vi "PicoScope5000aOpen.vi"(0 "error in (no error)":errorcluster, 1 "Serial Number":string, 2 "Mode":u16(ring) items=["Dialog On Error", "no dialog - CloseUnit and Stop", "no dialog - Continue", "no dialog - Stop"], 5 "Use Serial Number":bool, 9 "Resolution":u32(ring) items=["8-bit", "12-bit", "14-bit", "15-bit (max. 2 ch.)", "16-bit (max. 1 ch.)"], 11 "USB Powered control":bool=TRUE, 15 "USB 3.0 device on non-USB 3.0 Port control":bool=TRUE) -> (3 "USB 3.0 device on non-USB 3.0 Port":bool=TRUE, 4 "error out":errorcluster, 6 "handle":i16, 10 "USB Powered":bool=TRUE, 12 "Device Info":T1, 14 "Max ADC value":i16)   [LabVIEW 2010]
doc: "This VI opens a PicoScope ps5000a API device and returns a handle to the device."
uses:
  ps5000a.dll
panel:
  out "count":i16
  out "serialLth":i16
  out "Pico 5000a Units":string
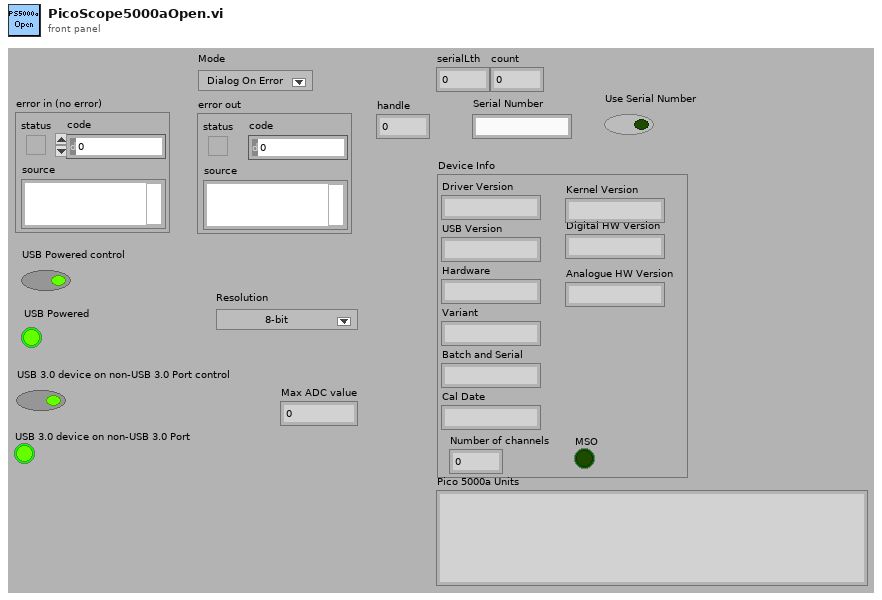
[diagram p1: front panel]
types:
  T1 = cluster{"Driver Version":string, "USB Version":string, "Hardware":string, "Variant":string, "Batch and Serial":string, "Cal Date":string, "Kernel Version":string, "Digital HW Version":string, "Analogue HW Version":string, "MSO":bool, "Number of channels":i16}
  T2 = cluster{"status":bool, "code":u32, "source":string}
  T3 = cluster{"Driver Version":string, "USB Version":string, "Hardware":string, "Variant":string, "Batch and Serial":string, "Cal Date":string, "Kernel Version":string, "Digital HW Version":string, "Analogue HW Version":string, "Firmware 1":string, "Firmware 2":string}
  T4 = cluster{"Driver Version":string, "USB Version":string, "Hardware":string, "Variant":string, "Batch and Serial":string, "Cal Date":string, "Kernel Version":string, "Digital HW Version":string, "Analogue HW Version":string, bool, i16}
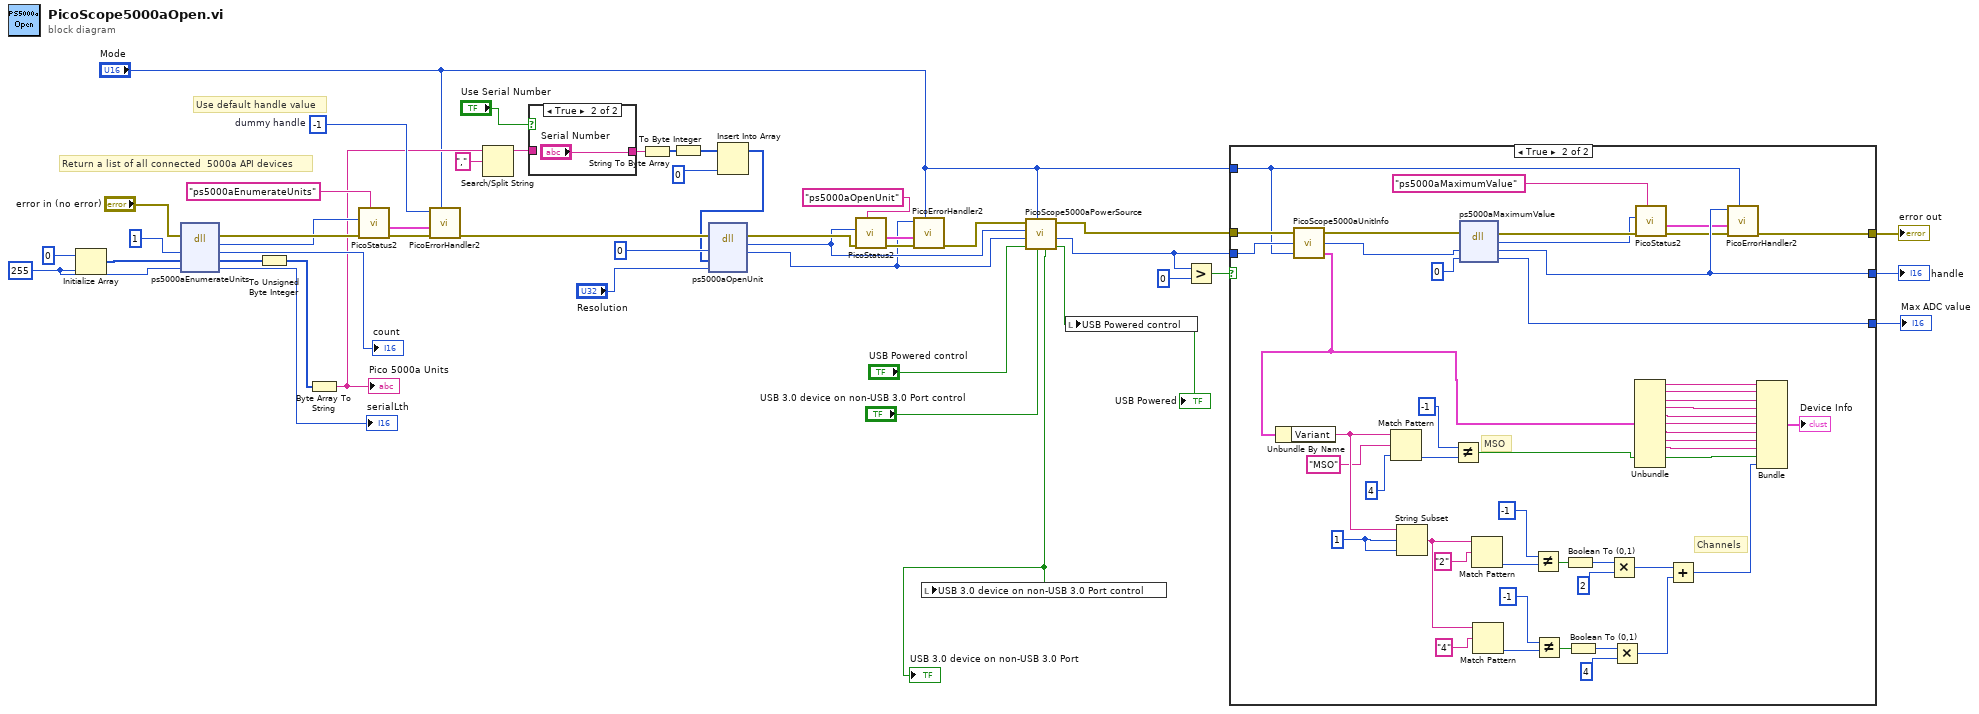
[diagram p0: block diagram]
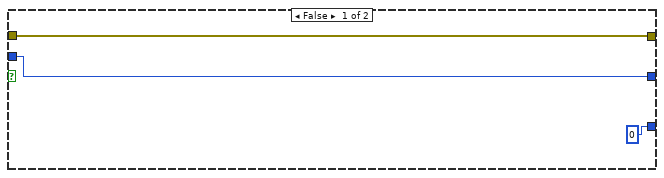
[diagram p3: hidden frame]
diagram:
  w26 = i16 -1  # dummy handle
  w29 = i16 255 ("dimension size")
  # "Use default handle value"
  # "Return a list of all connected  5000a API devices"
  n1 = Initialize Array(i8 0 ("U8"), w29) -> (w31:i8[])
  n2 = dll-call lib="ps5000a.dll" fn="ps5000aEnumerateUnits"(error in="error in (no error)", "count"=i16 1, "serials"=w31, "serialLth"=w29) -> (error out=w23:errorcluster, "PICO_STATUS"=w21:u32, "count"=→"count":i16, "serials"=w27:i8[], "serialLth"=→"serialLth":i16)  [unwired: 2 in, 1 out]
  n3 = To Unsigned Byte Integer(number=w27) -> (unsigned 8bit integer=w28:u8[])
  n4 = Byte Array To String(unsigned byte array=w28) -> (string=w15:string)
  "Pico 5000a Units" <- w15
  n5 = call "PicoStatus2.vi"("PICO source"="ps5000aEnumerateUnits" ("source"), "Error in"=w23, "PICO STATUS"=w21) -> ("error out"=w25:errorcluster, "PICO_STATUS out"=w24:T2)  [unwired: 5 in]
  n6 = call "PicoErrorHandler2.vi"("Mode"="Mode", "error in (no error)"=w25, "PICO_STATUS in"=w24, "handle In"=w26) -> ("error out"=w35:errorcluster)  [unwired: 7 in]
  n7 = Search/Split String(string=w15, search string/char (-)=",") -> (substring before match=w13:string)  [unwired: 1 in, 2 out]
  n8 = case shown="True" "Use Serial Number" {
    tunnel: w13 -> [w47 _]
    tunnel: [w47 "Serial Number"] -> w9
    frame False {
    }
    frame True {
    }
  }
  n9 = String To Byte Array(string=w9) -> (unsigned byte array=w11:u8[])
  n10 = To Byte Integer(number=w11) -> (8bit integer=w12:i8[])
  n11 = Insert Into Array(array=w12, new element=i8 0 ("new element/subarray")) -> (w8:i8[])  [unwired: 1 in]
  n12 = dll-call lib="ps5000a.dll" fn="ps5000aOpenUnit" ("ps3000.dll:_ps3000_open_unit@0")(error in=w35, "handle"=i16 0, "serial"=w8, "resolution"="Resolution") -> (error out=w18:errorcluster, "PICO_STATUS"=w3:u32, "handle"=w2:i16)  [unwired: 4 in, 1 out]
  n13 = call "PicoStatus2.vi"("PICO source"="ps5000aOpenUnit" ("source"), "Error in"=w18, "PICO STATUS"=w3) -> ("error out"=w17:errorcluster, "PICO_STATUS out"=w20:T2)  [unwired: 5 in]
  n14 = call "PicoErrorHandler2.vi"("Mode"="Mode", "error in (no error)"=w17, "PICO_STATUS in"=w20, "handle In"=w2) -> ("error out"=w4:errorcluster)  [unwired: 7 in]
  n15 = call "PicoScope5000aPowerSource.vi"("USB 3.0 on non-USB 3.0 port control"="USB 3.0 device on non-USB 3.0 Port control", "Mode"="Mode", "USB Powered control"="USB Powered control", "handle in"=w2, "PICO STATUS IN"=w3, "error in (no error)"=w4) -> ("USB Powered"=w45:bool, "handle out"=w43:i16, "error out"=w38:errorcluster, "USB 3.0 on non-USB 3.0 Port"=w39:bool)  [unwired: 1 in, 1 out]
  "USB Powered" <- w45
  "USB 3.0 device on non-USB 3.0 Port" <- w39
  n16 = local write "USB 3.0 device on non-USB 3.0 Port control"(w39) -> ()
  n17 = local write "USB Powered control"(w45) -> ()
  n18 = Greater?(x=w43, y=0) -> (0:w44:bool)
  n19 = case shown="True" w44 {
    tunnel: w43 -> [w50 w99]
    tunnel: w38 -> [w51 w98]
    tunnel: [w51 w60] -> w36
    tunnel: [w50 w59] -> w37
    tunnel: [i16 0 ("value") w61] -> w41
    tunnel: "Mode" -> [_ w52]
    frame False {
    }
    frame True {
      w88 = 1 ("offset (0)")
      # "MSO"
      # "Channels"
      n20 = call "PicoScope5000aUnitInfo.vi"("Mode"=w52, "handle in"=w99, "error in (no error)"=w98) -> ("Unit Info"=w64:T3, "handle out"=w63:i16, "error out"=w54:errorcluster)
      n21 = Unbundle By Name(w64) -> ("Variant"=w84:string)
      n22 = Match Pattern(string=w84, regular expression="MSO", offset (0)=4) -> (offset past match=w81:i32)  [unwired: 3 out]
      n23 = String Subset(string=w84, offset (0)=w88, length (rest)=w88) -> (substring=w75:string)
      n24 = Not Equal?(x=-1, y=w81) -> (x != y?=w79:bool)
      n25 = dll-call lib="ps5000a.dll" fn="ps5000aMaximumValue"(error in=w54, "handle"=w63, "value"=i16 0) -> (error out=w57:errorcluster, "PICO_STATUS"=w55:u32, "handle"=w59:i16, "value"=w61:i16)  [unwired: 2 in, 1 out]
      n26 = Match Pattern(string=w75, regular expression="2") -> (offset past match=w86:i32)  [unwired: 1 in, 3 out]
      n27 = Match Pattern(string=w75, regular expression="4") -> (offset past match=w77:i32)  [unwired: 1 in, 3 out]
      n28 = Not Equal?(x=-1, y=w86) -> (x != y?=w71:bool)
      n29 = Not Equal?(x=-1, y=w77) -> (x != y?=w67:bool)
      n30 = Boolean To (0,1)(Boolean=w71) -> (0, 1=w70:i16)
      n31 = Boolean To (0,1)(Boolean=w67) -> (0, 1=w68:i16)
      n32 = Multiply(x=w70, y=i16 2) -> (x*y=w74:i16)
      n33 = Multiply(x=w68, y=i16 4) -> (x*y=w66:i16)
      n34 = Unbundle(w64) -> ("Driver Version"=w97:string, "USB Version"=w96:string, "Hardware"=w95:string, "Variant"=w94:string, "Batch and Serial"=w93:string, "Cal Date"=w92:string, "Kernel Version"=w91:string, "Digital HW Version"=w90:string, "Analogue HW Version"=w89:string)  [unwired: 2 out]
      n35 = call "PicoStatus2.vi"("PICO source"="ps5000aMaximumValue" ("source"), "Error in"=w57, "PICO STATUS"=w55) -> ("error out"=w58:errorcluster, "PICO_STATUS out"=w56:T2)  [unwired: 5 in]
      n36 = Add(x=w74, y=w66) -> (x+y=w73:i16)
      n37 = call "PicoErrorHandler2.vi"("Mode"=w52, "error in (no error)"=w58, "PICO_STATUS in"=w56, "handle In"=w59) -> ("error out"=w60:errorcluster)  [unwired: 7 in]
      n38 = Bundle("Driver Version"=w97, "USB Version"=w96, "Hardware"=w95, "Variant"=w94, "Batch and Serial"=w93, "Cal Date"=w92, "Kernel Version"=w91, "Digital HW Version"=w90, "Analogue HW Version"=w89, w79, w73) -> (→"Device Info":T4)  [unwired: 1 in]
    }
  }
  "handle" <- w37
  "error out" <- w36
  "Max ADC value" <- w41
